vi "Sous_VI_Virage_1.vi"() -> ()   [LabVIEW 2017]
panel:
  out "x > y ? 3":bool[](array[boolean])
  out "x > y ? 2":bool[](array[boolean])
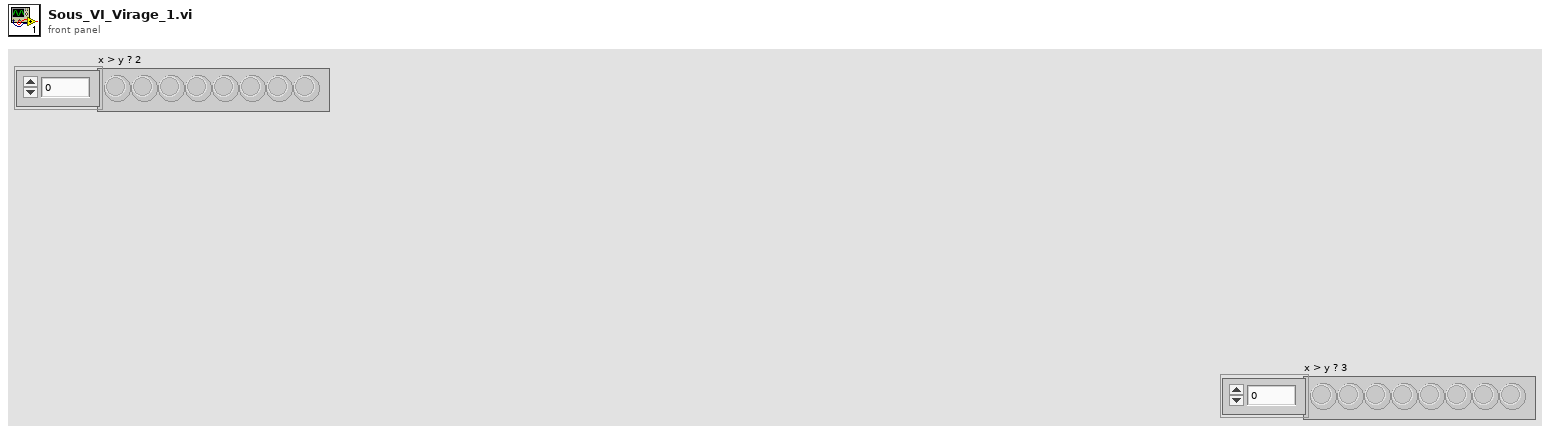
[diagram p1: front panel]
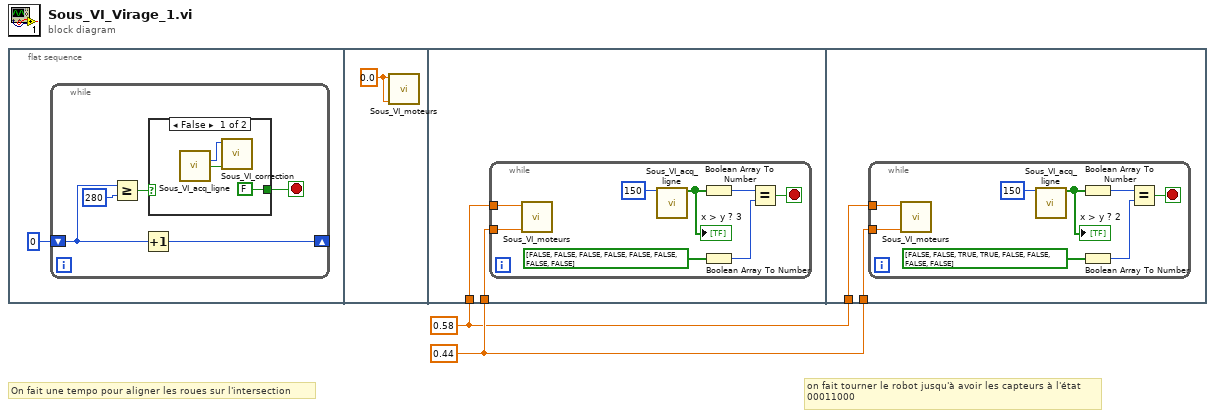
[diagram p0: block diagram]
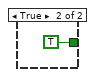
[diagram p2: hidden frame]
diagram:
  w1 = 0.58 ("moteur gauche vite")
  w2 = 0.44 ("moteur droit lent")
  # "on fait tourner le robot jusqu'à avoir les capteurs à l'état\n00011000"
  # "On fait une tempo pour aligner les roues sur l'intersection"
  n1 = flat-sequence {
    tunnel: w2 -> [w15]
    tunnel: w1 -> [w14]
    tunnel: w1 -> [w25]
    tunnel: w2 -> [w24]
    frame #0 {
      n2 = while {
        shift-right: [w8] -> _
        shift-left: 0 -> [w5]
        stop <- w6 stop-if-true
        n3 = Greater Or Equal?(x=w5, y=280) -> (x >= y?=w7:bool)
        n4 = Increment(x=w5) -> (x+1=w8:i32)
        n5 = case shown="False" w7 {
          tunnel: [FALSE TRUE] -> w6
          frame False {
            n6 = call "Sous_VI_acq_ligne.vi"() -> ("Décalage"=w10:u32, "G/D ?"=w9:bool)  [unwired: 11 in, 3 out]
            n7 = call "Sous_VI_correction.vi"("G/D ?"=w9, "Décalage"=w10) -> ()  [unwired: 10 in]
          }
          frame True {
          }
        }
      }
    }
    frame #1 {
      w13 = 0.0 ("Moteur Gauche")
      n8 = call "Sous_VI_moteurs.vi"("Moteur Droit"=w13, "Moteur Gauche"=w13) -> ()  [unwired: 10 in]
    }
    frame #2 {
      n9 = while {
        tunnel: w14 -> [w18]
        tunnel: w15 -> [w19]
        stop <- w20 stop-if-true
        n10 = call "Sous_VI_moteurs.vi"("Moteur Droit"=w19, "Moteur Gauche"=w18) -> ()  [unwired: 10 in]
        n11 = call "Sous_VI_acq_ligne.vi"("Seuil"=150) -> ("x > y ?"=w17:bool[])  [unwired: 10 in, 4 out]
        "x > y ? 3" <- w17
        n12 = Boolean Array To Number(Boolean array=w17) -> (number=w21:u32)
        n13 = Boolean Array To Number(Boolean array=bool[] [FALSE, FALSE, FALSE, FALSE, FALSE, FALSE, FALSE, FALSE]) -> (number=w22:u32)
        n14 = Equal?(x=w21, y=w22) -> (x = y?=w20:bool)
      }
    }
    frame #3 {
      n15 = while {
        tunnel: w25 -> [w28]
        tunnel: w24 -> [w29]
        stop <- w30 stop-if-true
        n16 = call "Sous_VI_moteurs.vi"("Moteur Droit"=w29, "Moteur Gauche"=w28) -> ()  [unwired: 10 in]
        n17 = call "Sous_VI_acq_ligne.vi"("Seuil"=150) -> ("x > y ?"=w27:bool[])  [unwired: 10 in, 4 out]
        "x > y ? 2" <- w27
        n18 = Boolean Array To Number(Boolean array=w27) -> (number=w31:u32)
        n19 = Boolean Array To Number(Boolean array=bool[] [FALSE, FALSE, TRUE, TRUE, FALSE, FALSE, FALSE, FALSE]) -> (number=w32:u32)
        n20 = Equal?(x=w31, y=w32) -> (x = y?=w30:bool)
      }
    }
  }
